vi "Test String Length.vi"(8 "error in (no error)":errorcluster) -> (0 "error out":errorcluster, 3 "Pass?":bool)   [LabVIEW 2020]
uses:
  G-Unicode/Types/UTF-8 String/UTF-8 String.lvclass/UTF-8 String.ctl
  afc09de1-d9a4-4e26-9d52-ac1d88bb7c1d.vi
  b0f689db-263b-41ba-8052-3b219af6c750.vi
  G-Unicode/Private/Conversion/String as Encoded String.vi
  G-Unicode/Private/Conversion/Polymorphic VIs/String as Encoded String (UTF-8 String).vi
  G-Unicode/Private/Conversion/Polymorphic VIs/String as Encoded String (LabVIEW String).vi
  G-Unicode/Types/UTF-8 String/Read Encoded UTF-8 String.vi
  G-Unicode/Private/Conversion/Text to UTF-8.vi
  G-Unicode/Private/Conversion/Polymorphic VIs/Text to UTF-8 (LabVIEW String).vi
  G-Unicode/Private/Library/gu_strlen.vi
  G-Unicode/Types/UTF-8 String/UTF-8 String.lvclass
  b26c07e1-af0a-4265-8363-a2494f47ceb2.vi
  G-Unicode/Unicode/Controls/String Encoding.ctl
  G-Unicode/G-Unicode.lvlib
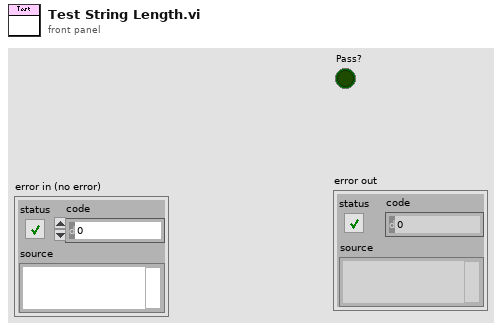
[diagram p1: front panel]
types:
  T1 = typedef "G-Unicode.lvlib/String Encoding.ctl" = enum16{"ANSI", "UTF-8", "UTF-16LE", "UTF-16BE", "Unknown"}
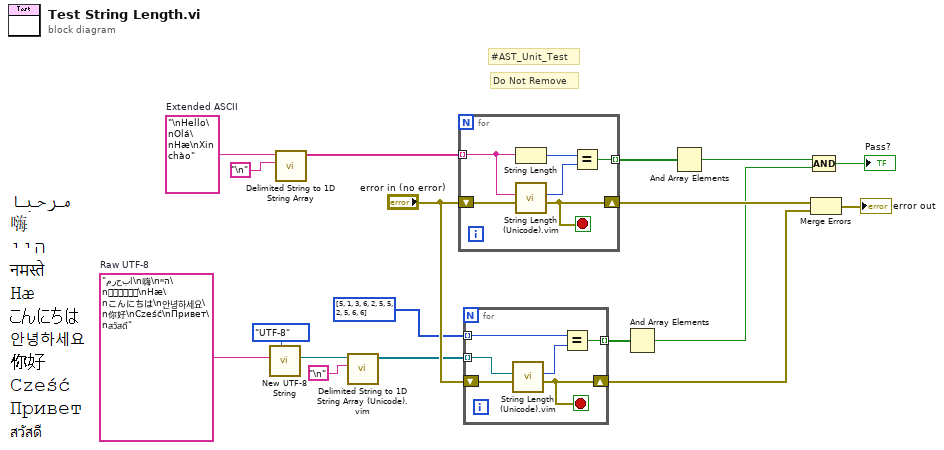
[diagram p0: block diagram]
diagram:
  w8 = "\nHello\nOlá\nHæ\nXin chào"  # Extended ASCII
  w2 = "مرحبا\n嗨\nהיי\nनमस्ते\nHæ\nこんにちは\n안녕하세요\n你好\nCześć\nПривет\nสวัสดี"  # Raw UTF-8
  # "Do Not Remove"
  # "#AST_Unit_Test"
  n1 = call "New UTF-8 String.vi"("Input Encoding (ANSI)"=String_Encoding."UTF-8", "String"=w2) -> ("UTF-8 String"=w4:refnum<class "UTF-8 String.lvclass">)  [unwired: 8 in, 1 out]
  n2 = call <vilib>:"Delimited String to 1D String Array.vi"("delimiter"="\n", "delimited string"=w8) -> ("string array"=w7:string[])  [unwired: 9 in]
  n3 = call "Delimited String to 1D String Array (Unicode).vim"("Delimiter (tab)"="\n", "Delimited String"=w4) -> ("String Array"=w1:refnum<class "UTF-8 String.lvclass">[])  [unwired: 8 in, 1 out]
  n4 = for {
    tunnel: [w24] -> w15 mode=indexing
    shift-right: [w19] -> w18
    shift-left: "error in (no error)" -> [w22]
    tunnel: w7 -> [w21] mode=indexing
    stop <- w19 stop-if-true
    n5 = String Length(string=w21) -> (length=w23:i32)
    n6 = call "String Length (Unicode).vim"("error in"=w22, "String"=w21) -> ("error out"=w19:errorcluster, "Length"=w20:i32)  [unwired: 8 in]
    n7 = Equal?(x=w23, y=w20) -> (x = y?=w24:bool)
  }
  n8 = for {
    tunnel: w1 -> [w28] mode=indexing
    tunnel: [w30] -> w13 mode=indexing
    shift-right: [w26] -> w11
    shift-left: "error in (no error)" -> [w27]
    tunnel: i32[] [5, 1, 3, 6, 2, 5, 5, 2, 5, 6, 6] ("Array") -> [w29] mode=indexing
    stop <- w26 stop-if-true
    n9 = call "String Length (Unicode).vim"("error in"=w27, "String"=w28) -> ("error out"=w26:errorcluster, "Length"=w25:i32)  [unwired: 8 in]
    n10 = Equal?(x=w29, y=w25) -> (x = y?=w30:bool)
  }
  n11 = And Array Elements(Boolean array=w13) -> (logical AND=w12:bool)
  n12 = And Array Elements(Boolean array=w15) -> (logical AND=w14:bool)
  n13 = Merge Errors(w18, w11) -> (→"error out":errorcluster)
  n14 = Compound Arithmetic op=AND(w14, w12) -> (→"Pass?":bool)
